vi "Configure Websockets Connection.vi"(4 "Read Mode (Immediate)":T1(ring)=enum."Immediate", 5 "Connection.Websockets":refnum<class "Connection.WS.lvclass">, 6 "timeout (5000ms)":i32=5000, 7 "path (/)":string="/", 8 "error in (no error)":errorcluster, 9 "subProtocols":string[](array[string]), 10 "remote port (80)":u16=80, 11 "address (localhost)":string="localhost") -> (0 "error out":errorcluster, 3 "Connection.Websockets":refnum<class "Connection.WS.lvclass">)   [LabVIEW 2013, in "Connection.WS_GOSPL.lvlib" / "Connection.WS.lvclass"]
uses:
  Connection.WS.lvclass
  Connection.TCP/Connection.TCP.lvclass/Connection.TCP.ctl
  Connection.WS.lvclass/Connection.WS.ctl
  Connection/Connection.lvclass/Connection.ctl
  Connection/Connection.lvclass
  Connection.TCP/Connection.TCP.lvclass
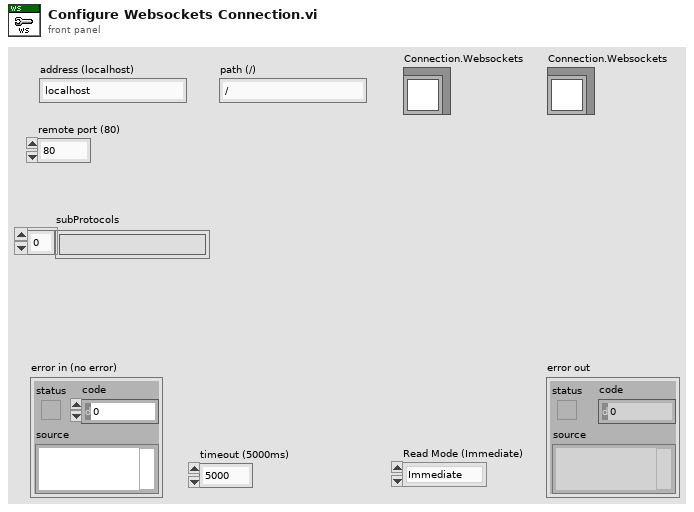
[diagram p1: front panel]
types:
  T1 = enum16{"Standard", "Buffered", "CRLF", "Immediate"}
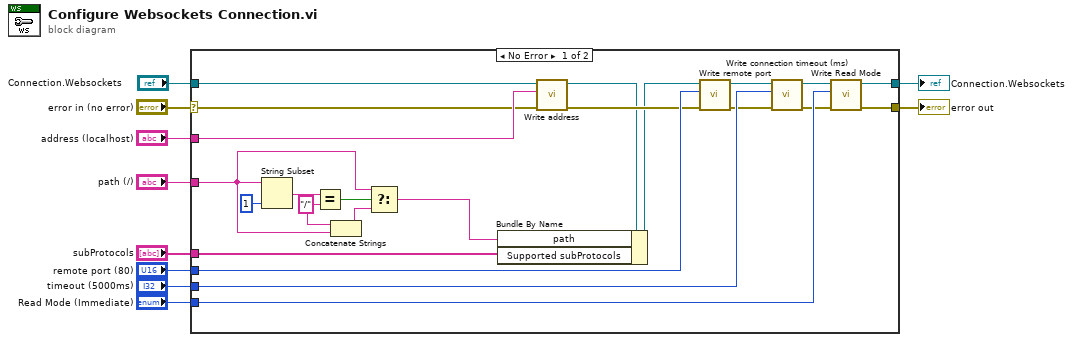
[diagram p0: block diagram]
diagram:
  n1 = case shown="No Error" "error in (no error)" {
    selector: "error in (no error)" -> [w21 w35]
    tunnel: [w25 w35] -> w9
    tunnel: [w27 w34] -> w5
    tunnel: "address (localhost)" -> [w30 _]
    tunnel: "remote port (80)" -> [w32 _]
    tunnel: "timeout (5000ms)" -> [w33 _]
    tunnel: "Read Mode (Immediate)" -> [w26 _]
    tunnel: "Connection.Websockets" -> [w31 w34]
    tunnel: "path (/)" -> [w12 _]
    tunnel: "subProtocols" -> [w18 _]
    frame No Error {
      w14 = "/" ("y")
      n2 = String Subset(string=w12, length (rest)=1 ("length (rest)")) -> (substring=w16:string)  [unwired: 1 in]
      n3 = Equal?(x=w16, y=w14) -> (x = y?=w15:bool)
      n4 = Concatenate Strings(w14, w12) -> (w13:string)
      n5 = Select(t=w12, s=w15, f=w13) -> (s? t:f=w11:string)
      n6 = call "Write address.vi"("error in (no error)"=w21, "address"=w30, "Connection.TCP"=w31) -> ("error out"=w22:errorcluster, "Connection.TCP"=w20:refnum<class "Connection.WS.lvclass">)  [unwired: 7 in]
      n7 = Bundle By Name(cluster=w20, "path"=w11, "Supported subProtocols"=w18) -> (w19:refnum<class "Connection.WS.lvclass">)
      n8 = call "Write remote port.vi"("error in (no error)"=w22, "remote port (80)"=w32, "Connection.TCP"=w19) -> ("error out"=w23:errorcluster, "Connection.TCP"=w29:refnum<class "Connection.WS.lvclass">)  [unwired: 7 in]
      n9 = call "Write connection timeout (ms).vi"("error in (no error)"=w23, "connection timeout (ms)"=w33, "Connection in"=w29) -> ("error out"=w24:errorcluster, "Connection out"=w28:refnum<class "Connection.WS.lvclass">)  [unwired: 7 in]
      n10 = call "Write Read Mode.vi"("error in (no error)"=w24, "Read Mode"=w26, "Connection.TCP"=w28) -> ("error out"=w25:errorcluster, "Connection.TCP"=w27:refnum<class "Connection.WS.lvclass">)  [unwired: 7 in]
    }
    frame Error {
    }
  }
  "error out" <- w9
  "Connection.Websockets" <- w5
